vi "Welcome.vi"() -> ()   [LabVIEW 2021]
panel:
  in  "stop":bool
  in  "String":string
  # "BIENVENUE AU PROGRAMME DU CENTRE D'APPELS !"
  # "Entrez votre nom"
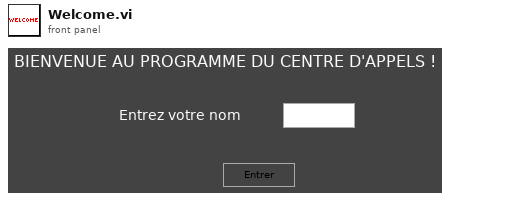
[diagram p1: front panel]
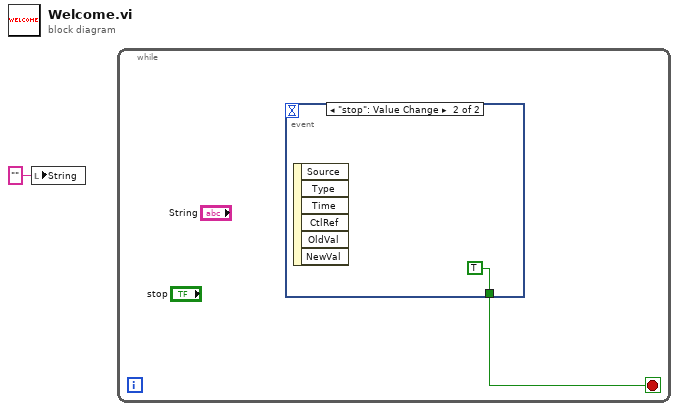
[diagram p0: block diagram]
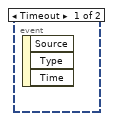
[diagram p2: hidden frame]
diagram:
  n1 = local write "String"("" ("String")) -> ()
  n2 = while {
    stop <- w2 stop-if-true
    n3 = event shown="[1] \"stop\": Value Change" {
      selector: _ -> [_ _]
      dyn-events: _ -> [_ _]
      timeout: _ -> [_ _]
      tunnel: [_ TRUE] -> w2
      event Timeout {
        n4 = event-data() -> ()  [unwired: 1 in, 3 out]
      }
      event "stop": Value Change {
        n5 = event-data() -> ()  [unwired: 1 in, 6 out]
      }
    }
  }
